vi "Tear Down TS.vi"(8 "error in":errorcluster, 11 "DeepU Test Stand in":refnum<class "DeepU Test Stand.lvclass">) -> (0 "error out":errorcluster, 3 "DeepU Test Stand out":refnum<class "DeepU Test Stand.lvclass">)   [LabVIEW 2019, in "Test Stands.lvlib" / "DeepU Test Stand.lvclass"]
uses:
  DeepU Test Stand.lvclass
  <vilib>/DAQmx/write.llb/DAQmx Write (Digital Bool 1Line 1Point).vi
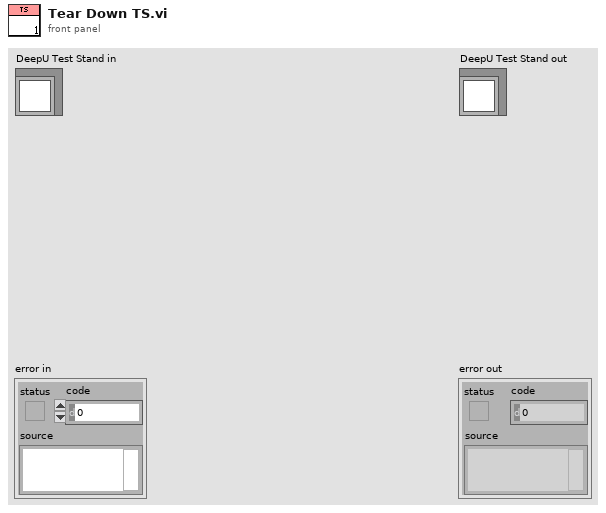
[diagram p1: front panel]
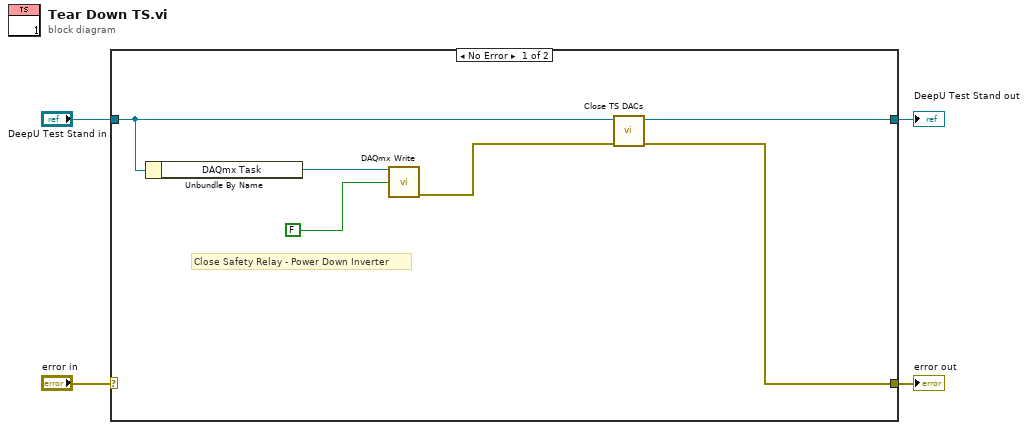
[diagram p0: block diagram]
diagram:
  n1 = case shown="No Error" "error in" {
    selector: "error in" -> [_ w12]
    tunnel: [w9 w12] -> w4
    tunnel: [w10 w11] -> w3
    tunnel: "DeepU Test Stand in" -> [w8 w11]
    frame No Error {
      # "Close Safety Relay - Power Down Inverter"
      n2 = Unbundle By Name(w8) -> ("DAQmx Task"=w6:refnum<k21>)
      n3 = call-poly <vilib>:"DAQmx Write.vi"("task/channels in"=w6, "data"=FALSE) -> ("error out"=w5:errorcluster)  [unwired: 11 in, 2 out]
      n4 = call "Close TS DACs.vi"("error in (no error)"=w5, "DeepU Test Stand in"=w8) -> ("error out"=w9:errorcluster, "DeepU Test Stand out"=w10:refnum<class "DeepU Test Stand.lvclass">)  [unwired: 8 in]
    }
    frame Error {
    }
  }
  "error out" <- w4
  "DeepU Test Stand out" <- w3
